vi "Migrate - Backup INI Files.vi"(8 "error in (no error)":errorcluster, 11 "Data Folder":path) -> (0 "error out":errorcluster, 3 "Backup Folder":path)   [LabVIEW 2024]
doc: "Copies every *.ini file of the data folder into a new subfolder Backup v1 YYYY-MM-DD HHMMSS (local time) and returns its path. Any failure - the folder cannot be created or a file cannot be copied - is returned as an error, so the caller can abort before it changes anything.\n\nGenerated by: Claude"
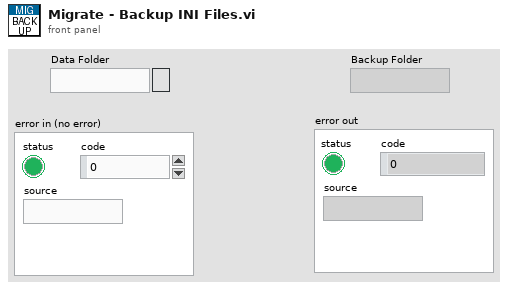
[diagram p1: front panel]
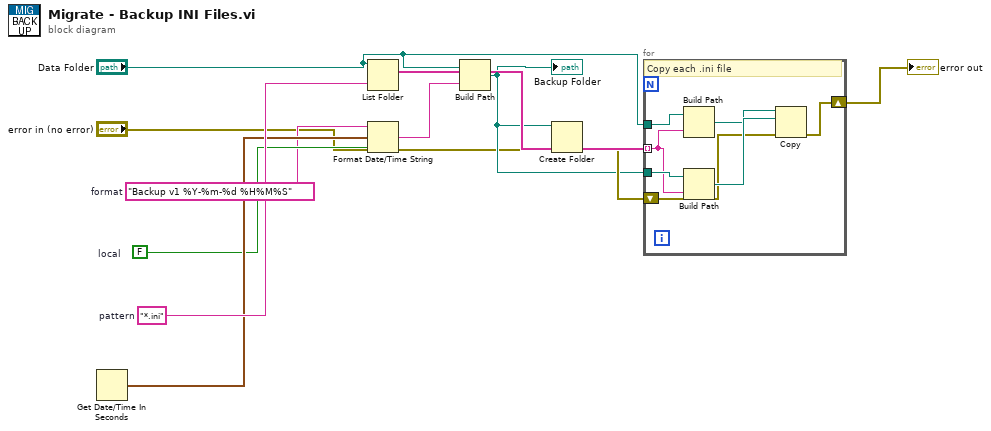
[diagram p0: block diagram]
diagram:
  w9 = "*.ini"  # pattern
  w4 = FALSE  # local
  w3 = "Backup v1 %Y-%m-%d %H%M%S"  # format
  n1 = Get Date/Time In Seconds() -> (seconds since 1Jan1904=w5:timestamp)
  n2 = List Folder(path="Data Folder", pattern=w9) -> (filenames=w10:string[])  [unwired: 2 in, 3 out]
  n3 = Format Date/Time String(time format string (%c)=w3, seconds (now)=w5, UTC format=w4) -> (date/time string=w6:string)
  n4 = Build Path(base path="Data Folder", name or relative path=w6) -> (appended path=w7:path)
  "Backup Folder" <- w7
  n5 = Create Folder(path (use dialog)=w7, error in="error in (no error)") -> (error out=w8:errorcluster)  [unwired: 1 in, 2 out]
  n6 = for {
    tunnel: "Data Folder" -> [w13]
    tunnel: w10 -> [w12] mode=indexing
    tunnel: w7 -> [w14]
    shift-right: [w16] -> w11
    shift-left: w8 -> [w15]
    # "Copy each .ini file"
    n7 = Build Path(base path=w13, name or relative path=w12) -> (appended path=w17:path)
    n8 = Build Path(base path=w14, name or relative path=w12) -> (appended path=w18:path)
    n9 = Copy(8:w15, 10:w18, 11:w17) -> (0:w16:errorcluster)  [unwired: 2 in, 2 out]
  }
  "error out" <- w11
